vi "Duplicate Name Error Test.vi"() -> (0 "error out":errorcluster, 1 "Success Error on Replace Line":bool, 2 "Success Error on Write Lines":bool, 3 "Success Error on Add":bool)   [LabVIEW 2015, in "DAQmx Module Tests.lvlib"]
doc: "Tests the Add Line and Remove Line functions."
uses:
  DAQmx Module Tests.lvlib
  module/configuration/Line.ctl
  <vilib>/NI/Tag Bus Module Framework/channel/TBM channel.lvclass
  module/configuration/Measurement Type.ctl
  module/configuration/Parameters.ctl
  module/configuration/Get Line Name.vi
  <vilib>/NI/Tag Bus Module Framework/module configuration/FindDuplicate.vi
  <vilib>/Utility/error.llb/Error Cluster From Error Code.vi
  module/configuration/Daqmx Module configuration.lvclass
  editor node/DAQmx Module editor node.lvclass
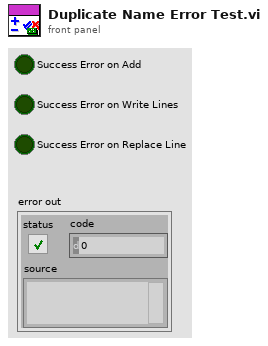
[diagram p1: front panel]
types:
  T1 = typedef "DAQmx Module Configuration.lvclass/Measurement Type.ctl" = enum16{"Digital Input", "Digital Output", "Voltage Input", "Voltage Output", "Current Input", "Current Output", "RTD", "Thermocouple", "Strain", "PWM"}
  T2 = typedef "DAQmx Module Configuration.lvclass/Line.ctl" = cluster{"Channel Array":refnum<class "TBM channel.lvclass">[], "Physical Channel":string, "Measurement Type":T1, "Parameters":T3}
  T3 = typedef "DAQmx Module Configuration.lvclass/Parameters.ctl" = cluster{"Digital Config":cluster{"Invert Lines?":bool}, "Voltage Config":cluster{"Maximum Value (V)":dbl, "Minimum Value (V)":dbl, "in terminal configuration (V)":i32, "out terminal configuration (V)":i32}, "Current Config":cluster{"Maximum Value (A)":dbl, "Minimum Value (A)":dbl, "shunt resistor location":i32, "input terminal configuration (C)":i32, "external shunt resistor value":dbl}, "RTD Config":cluster{"Maximum Value (°C)":dbl, "Minimum Value (°C)":dbl, "resistance configuration":i32, "r0":dbl, "current excitation value":dbl, "rtd type":i32, "current excitation source":i32}, "Thermocouple Config":cluster{"Minimum Value (C)":dbl, "Maximum Value (C)":dbl, "thermocouple type":i32, "cjc source":i32, "cjc value":dbl}, "Strain Config":cluster{"Maximum Value":dbl, "Minimum Value":dbl, "bridge information":cluster{"strain configuration":i32, "lead wire resistance":dbl, "initial bridge voltage":dbl, "voltage excitation source":i32, "voltage excitation value":dbl}, "strain gage information":cluster{"gage factor":dbl, "nominal gage resistance":dbl, "poisson ratio":dbl}}, "PWM Config":cluster{"Idle State":bool}}
  T4 = typedef "TBM channel.lvclass/channel classification.ctl" = enum16{"input data", "output data", "processing parameter", "processing result"}
  T5 = typedef "tag bus.lvlib/tag descriptor.lvclass/Data Type.ctl" = enum16{"Double", "Single", "I64", "I32", "I16", "I8", "U64", "U32", "U16", "U8", "Boolean", "String", "Array of Double", "Array of Single", "Array of I64", "Array of I32", "Array of I16", "Array of I8", "Array of U64", "Array of U32", "Array of U16", "Array of U8", "Array of Boolean", "Array of String"}
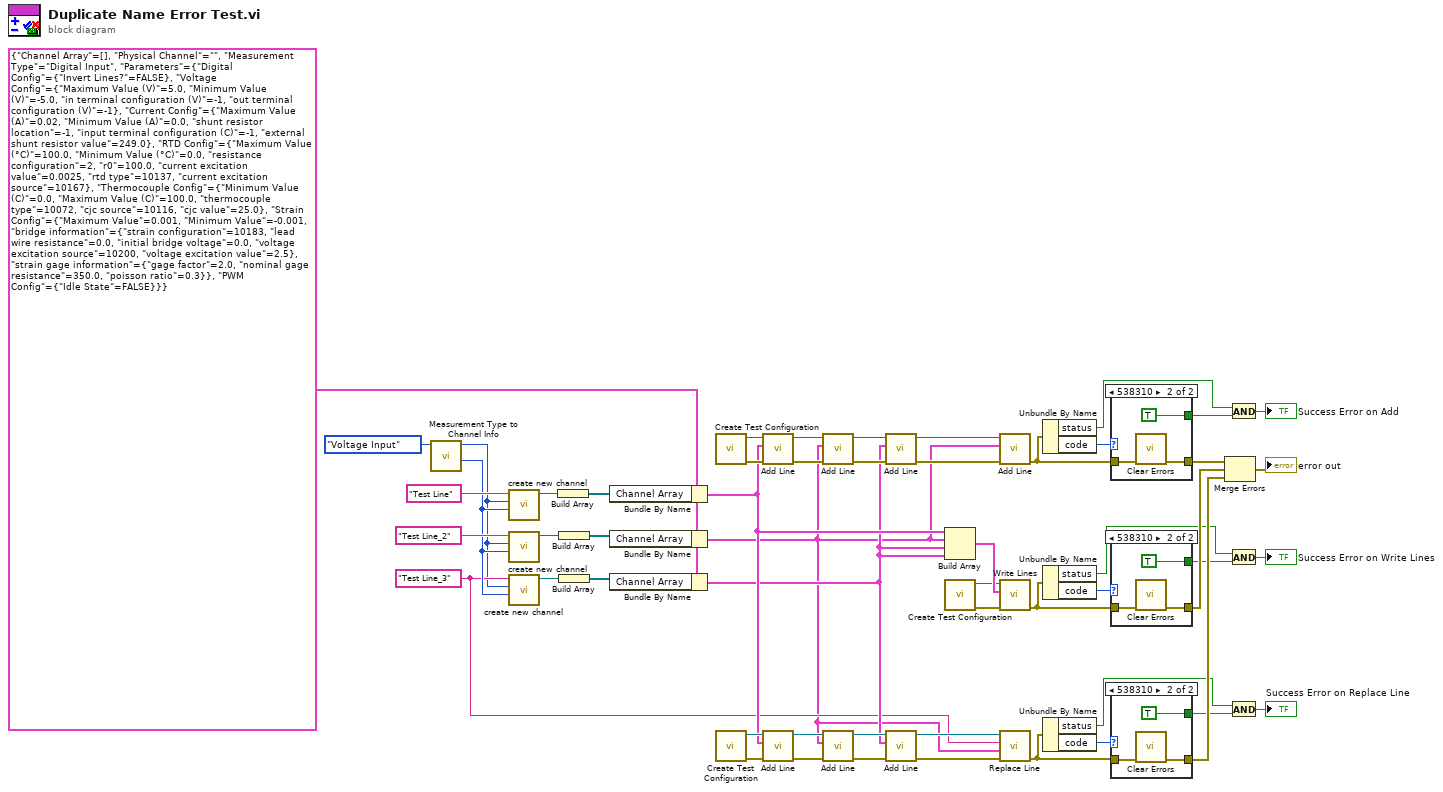
[diagram p0: block diagram]
diagram:
  w21 = "Test Line_3" ("channel name")
  w47 = T2 {"Channel Array"=[], "Physical Channel"="", "Measurement Type"=enum."Digital Input", "Parameters"={"Digital Config"={"Invert Lines?"=FALSE}, "Voltage Config"={"Maximum Value (V)"=5.0, "Minimum Value (V)"=-5.0, "in terminal configuration (V)"=-1, "out terminal configuration (V)"=-1}, "Current Config"={"Maximum Value (A)"=0.02, "Minimum Value (A)"=0.0, "shunt resistor location"=-1, "input terminal configuration (C)"=-1, "external shunt resistor value"=249.0}, "RTD Config"={"Maximum Value (°C)"=100.0, "Minimum Value (°C)"=0.0, "resistance configuration"=2, "r0"=100.0, "current excitation value"=0.0025, "rtd type"=10137, "current excitation source"=10167}, "Thermocouple Config"={"Minimum Value (C)"=0.0, "Maximum Value (C)"=100.0, "thermocouple type"=10072, "cjc source"=10116, "cjc value"=25.0}, "Strain Config"={"Maximum Value"=0.001, "Minimum Value"=-0.001, "bridge information"={"strain configuration"=10183, "lead wire resistance"=0.0, "initial bridge voltage"=0.0, "voltage excitation source"=10200, "voltage excitation value"=2.5}, "strain gage information"={"gage factor"=2.0, "nominal gage resistance"=350.0, "poisson ratio"=0.3}}, "PWM Config"={"Idle State"=FALSE}}} ("Line")
  n1 = call "Measurement Type to Channel Info.vi"("Measurement Type"=Measurement_Type."Voltage Input") -> ("channel classification"=w42:T4, "Data Type"=w5:T5)  [unwired: 8 in]
  n2 = call <vilib>:"create new channel.vi"("channel classification"=w42, "data type"=w5, "channel name"="Test Line") -> ("channel"=w53:refnum<class "TBM channel.lvclass">)  [unwired: 8 in]
  n3 = call <vilib>:"create new channel.vi"("channel classification"=w42, "data type"=w5, "channel name"="Test Line_2") -> ("channel"=w49:refnum<class "TBM channel.lvclass">)  [unwired: 8 in]
  n4 = call <vilib>:"create new channel.vi"("channel classification"=w42, "data type"=w5, "channel name"=w21) -> ("channel"=w48:refnum<class "TBM channel.lvclass">)  [unwired: 8 in]
  n5 = Build Array(w53) -> (w3:refnum<class "TBM channel.lvclass">[])
  n6 = Build Array(w49) -> (w2:refnum<class "TBM channel.lvclass">[])
  n7 = Build Array(w48) -> (w1:refnum<class "TBM channel.lvclass">[])
  n8 = Bundle By Name(cluster=w47, "Channel Array"=w3) -> (w24:T2)
  n9 = Bundle By Name(cluster=w47, "Channel Array"=w2) -> (w20:T2)
  n10 = Bundle By Name(cluster=w47, "Channel Array"=w1) -> (w23:T2)
  n11 = call "Create Test Configuration.vi"() -> ("error out"=w52:errorcluster, "Module Configuration"=w54:refnum<class "Daqmx Module configuration.lvclass">)  [unwired: 7 in, 3 out]
  n12 = call "Create Test Configuration.vi"() -> ("error out"=w26:errorcluster, "Module Configuration"=w25:refnum<class "Daqmx Module configuration.lvclass">)  [unwired: 7 in, 3 out]
  n13 = call "Add Line.vi"("error in"=w52, "Line"=w24, "Daqmx Module configuration in"=w54) -> ("error out"=w46:errorcluster, "Daqmx Module configuration out"=w43:refnum<class "Daqmx Module configuration.lvclass">)  [unwired: 6 in, 1 out]
  n14 = call "Add Line.vi"("error in"=w26, "Line"=w24, "Daqmx Module configuration in"=w25) -> ("error out"=w27:errorcluster, "Daqmx Module configuration out"=w30:refnum<class "Daqmx Module configuration.lvclass">)  [unwired: 6 in, 1 out]
  n15 = call "Add Line.vi"("error in"=w46, "Line"=w20, "Daqmx Module configuration in"=w43) -> ("error out"=w45:errorcluster, "Daqmx Module configuration out"=w44:refnum<class "Daqmx Module configuration.lvclass">)  [unwired: 6 in, 1 out]
  n16 = call "Add Line.vi"("error in"=w27, "Line"=w20, "Daqmx Module configuration in"=w30) -> ("error out"=w28:errorcluster, "Daqmx Module configuration out"=w29:refnum<class "Daqmx Module configuration.lvclass">)  [unwired: 6 in, 1 out]
  n17 = call "Add Line.vi"("error in"=w45, "Line"=w23, "Daqmx Module configuration in"=w44) -> ("error out"=w40:errorcluster, "Daqmx Module configuration out"=w41:refnum<class "Daqmx Module configuration.lvclass">)  [unwired: 6 in, 1 out]
  n18 = call "Add Line.vi"("error in"=w28, "Line"=w23, "Daqmx Module configuration in"=w29) -> ("error out"=w19:errorcluster, "Daqmx Module configuration out"=w22:refnum<class "Daqmx Module configuration.lvclass">)  [unwired: 6 in, 1 out]
  n19 = Build Array(w24, w20, w23, w23) -> (w37:T2[])
  n20 = call "Create Test Configuration.vi"() -> ("error out"=w18:errorcluster, "Module Configuration"=w36:refnum<class "Daqmx Module configuration.lvclass">)  [unwired: 7 in, 3 out]
  n21 = call "Add Line.vi"("error in"=w40, "Line"=w20, "Daqmx Module configuration in"=w41) -> ("error out"=w38:errorcluster)  [unwired: 6 in, 2 out]
  n22 = call "Write Lines.vi"("error in (no error)"=w18, "Lines"=w37, "Daqmx Module configuration in"=w36) -> ("error out"=w34:errorcluster)  [unwired: 7 in, 1 out]
  n23 = call "Replace Line.vi"("error in"=w19, "New Line"=w20, "Line Name"=w21, "Daqmx Module configuration in"=w22) -> ("error out"=w16:errorcluster)  [unwired: 5 in, 2 out]
  n24 = Unbundle By Name(w38) -> ("status"=w13:bool, "code"=w39:i32)
  n25 = Unbundle By Name(w34) -> ("status"=w8:bool, "code"=w35:i32)
  n26 = Unbundle By Name(w16) -> ("status"=w9:bool, "code"=w17:i32)
  n27 = case shown="538310" w39 {
    tunnel: w38 -> [w55 w58]
    tunnel: [w55 w57] -> w33
    tunnel: [_ TRUE ("Success Error on Add")] -> w14
    frame 0, Default {
    }
    frame 538310 {
      n28 = call <vilib>:"Clear Errors.vi"("error in (no error)"=w58) -> ("error out"=w57:errorcluster)  [unwired: 5 in, 1 out]
    }
  }
  n29 = case shown="538310" w35 {
    tunnel: w34 -> [w59 w62]
    tunnel: [w59 w61] -> w32
    tunnel: [_ TRUE ("Success Error on Add")] -> w7
    frame 0, Default {
    }
    frame 538310 {
      n30 = call <vilib>:"Clear Errors.vi"("error in (no error)"=w62) -> ("error out"=w61:errorcluster)  [unwired: 5 in, 1 out]
    }
  }
  n31 = case shown="538310" w17 {
    tunnel: w16 -> [w63 w66]
    tunnel: [w63 w65] -> w15
    tunnel: [_ TRUE ("Success Error on Add")] -> w10
    frame 0, Default {
    }
    frame 538310 {
      n32 = call <vilib>:"Clear Errors.vi"("error in (no error)"=w66) -> ("error out"=w65:errorcluster)  [unwired: 5 in, 1 out]
    }
  }
  n33 = Merge Errors(w33, w32, w15) -> (→"error out":errorcluster)
  n34 = And(x=w13, y=w14) -> (x .and. y?=→"Success Error on Add":bool)
  n35 = And(x=w8, y=w7) -> (x .and. y?=→"Success Error on Write Lines":bool)
  n36 = And(x=w9, y=w10) -> (x .and. y?=→"Success Error on Replace Line":bool)
